vi "Clear Connections.vi"(8 "error in (no error)":errorcluster, 11 "RT Data Cluster in":T1={"Timekeeper hdl"="", "clkDisc session"=variant, "Compiled Data"={"SyncMod?"=FALSE, "SyncMod"="", "ConnectionSettings"={"Mode"=enum."Generate sample clock", "pxitrig"=FALSE, "pfi0"=FALSE, "pfi1"=FALSE, "pfi2"=FALSE, "External Pin"=enum."PFI0", "Routes"=[]}, "TimeKeeper"="", "ScanOffset(%)"=0.0, "StartDelay(s)"=0, "Time Ref Settings"={"Time Reference"=enum."GPS", "Priority 1"=0, "Priority 2"=0, "IRIG type"=enum."IRIGB AM", "Terminal"="", "PPSSetTime"=FALSE, "Start Time"=timestamp(0 s since 1904-01-01)}, "FIFO Locations"={"BoardTime"=[], "Status"=[]}}, "OutputsData"=[], "OutputsFIFO"=refnum, "Scan Period"=0, "Timekeeper type"=enum."6683", "SyncMod type"=enum."6683", "SyncMod hdl"="", "Custom Device Name"=""} {"Compiled Data"."Time Ref Settings"."Priority 2" min=0 max=255; "Compiled Data"."Time Ref Settings"."Priority 1" min=0 max=255}) -> (0 "error out":errorcluster, 3 "RT Data Cluster out":T1={"Timekeeper hdl"="", "clkDisc session"=variant, "Compiled Data"={"SyncMod?"=FALSE, "SyncMod"="", "ConnectionSettings"={"Mode"=enum."Generate sample clock", "pxitrig"=FALSE, "pfi0"=FALSE, "pfi1"=FALSE, "pfi2"=FALSE, "External Pin"=enum."PFI0", "Routes"=[]}, "TimeKeeper"="", "ScanOffset(%)"=0.0, "StartDelay(s)"=0, "Time Ref Settings"={"Time Reference"=enum."GPS", "Priority 1"=0, "Priority 2"=0, "IRIG type"=enum."IRIGB AM", "Terminal"="", "PPSSetTime"=FALSE, "Start Time"=timestamp(0 s since 1904-01-01)}, "FIFO Locations"={"BoardTime"=[], "Status"=[]}}, "OutputsData"=[], "OutputsFIFO"=refnum, "Scan Period"=0, "Timekeeper type"=enum."6683", "SyncMod type"=enum."6683", "SyncMod hdl"="", "Custom Device Name"=""} {"Compiled Data"."Time Ref Settings"."Priority 2" min=0 max=255; "Compiled Data"."Time Ref Settings"."Priority 1" min=0 max=255})   [LabVIEW 2020, in "NI Synchronization Engine.lvlib"]
uses:
  NI Synchronization Engine.lvlib
  RT Data Cluster.ctl
  mdevClkDisc.llb/_clkDisc_session.ctl
  Shared/Compiled Data.ctl
  Shared/Connection Settings.ctl
  Shared/Mode.ctl
  Shared/External Pin.ctl
  Shared/Routes.ctl
  Shared/Route.ctl
  Shared/Time Ref Settings.ctl
  Shared/Time Reference.ctl
  Shared/IRIG Type.ctl
  timekeeper type.ctl
  Timekeeper Route Pin.ctl
  Shared/NI Synchronization Shared.lvlib
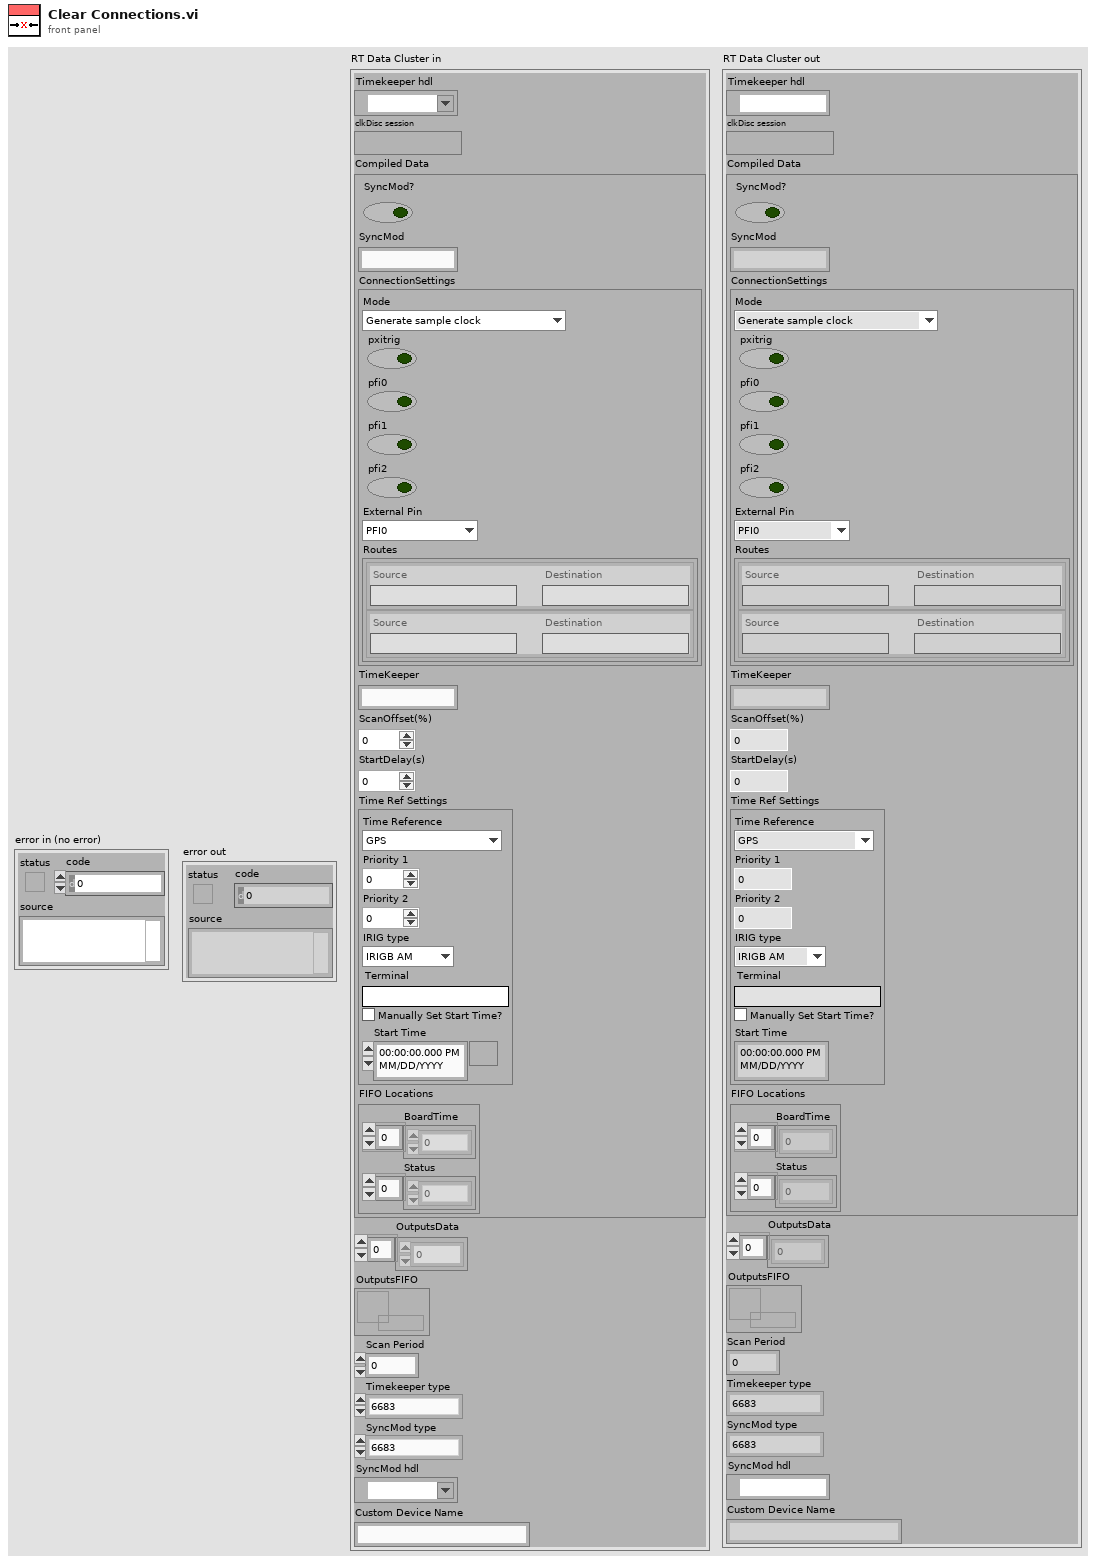
[diagram p1: front panel]
types:
  T1 = typedef "NI Synchronization Engine.lvlib/RT Data Cluster.ctl" = cluster{"Timekeeper hdl":refnum<k15>, "clkDisc session":T2, "Compiled Data":T3, "OutputsData":dbl[], "OutputsFIFO":refnum<k33>, "Scan Period":u32, "Timekeeper type":T12, "SyncMod type":T12, "SyncMod hdl":refnum<k15>, "Custom Device Name":string}
  T2 = typedef "_clkDisc_session.ctl" = variant
  T3 = typedef "NI Synchronization Shared.lvlib/Compiled Data.ctl" = cluster{"SyncMod?":bool, "SyncMod":string, "ConnectionSettings":T4, "TimeKeeper":string, "ScanOffset(%)":dbl, "StartDelay(s)":u16, "Time Ref Settings":T9, "FIFO Locations":cluster{"BoardTime":i32[], "Status":i32[]}}
  T4 = typedef "NI Synchronization Shared.lvlib/Connection Settings.ctl" = cluster{"Mode":T5, "pxitrig":bool, "pfi0":bool, "pfi1":bool, "pfi2":bool, "External Pin":T6, "Routes":T7}
  T5 = typedef "NI Synchronization Shared.lvlib/Mode.ctl" = enum16{"Generate sample clock", "Route sample clock out of chassis", "Route sample clock into chassis", "Custom routes"}
  T6 = typedef "NI Synchronization Shared.lvlib/External Pin.ctl" = enum16{"PFI0", "PFI1", "PFI2"}
  T7 = typedef "NI Synchronization Shared.lvlib/Routes.ctl" = T8[]
  T8 = typedef "NI Synchronization Shared.lvlib/Route.ctl" = cluster{"Source":string, "Destination":string}
  T9 = typedef "NI Synchronization Shared.lvlib/Time Ref Settings.ctl" = cluster{"Time Reference":T10, "Priority 1":i32, "Priority 2":i32, "IRIG type":T11, "Terminal":string, "PPSSetTime":bool, "Start Time":timestamp}
  T10 = typedef "NI Synchronization Shared.lvlib/Time Reference.ctl" = enum16{"GPS", "IRIG", "PPS", "1588 Ordinary Clock", "802.1AS", "PXI Chassis Clock", "Free Running (Internal)"}
  T11 = typedef "NI Synchronization Shared.lvlib/IRIG Type.ctl" = enum16{"IRIGB DC", "IRIGB AM"}
  T12 = typedef "NI Synchronization Engine.lvlib/timekeeper type.ctl" = enum16{"6683", "6683H", "6682", "6682H", "non-timekeeper", "timekeeper"}
  T13 = typedef "NI Synchronization Engine.lvlib/Timekeeper Route Pin.ctl" = enum16{"TTL0", "PFI0", "PFI1", "PFI2", "PXI_Clk10", "PXI_Clk10_In", "BoardClk", "ClkOut", "Oscillator"}
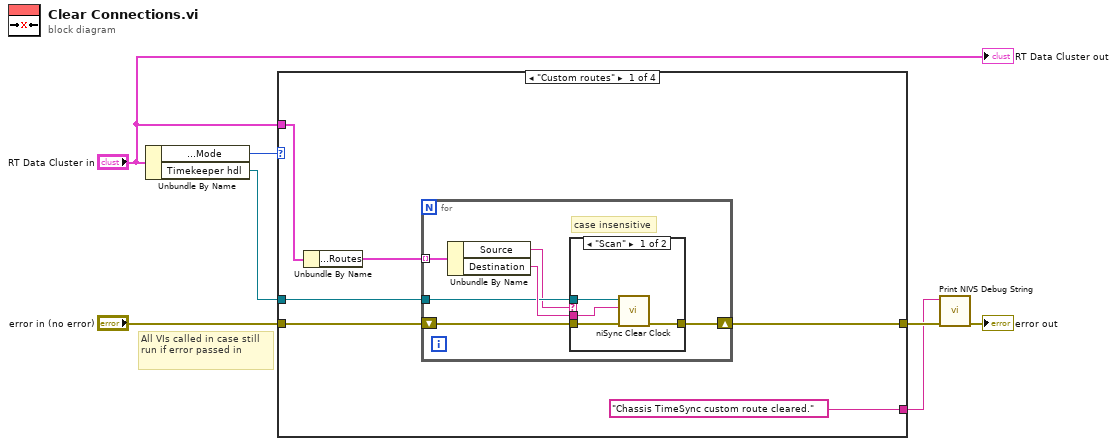
[diagram p0: block diagram]
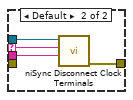
[diagram p2: hidden frame]
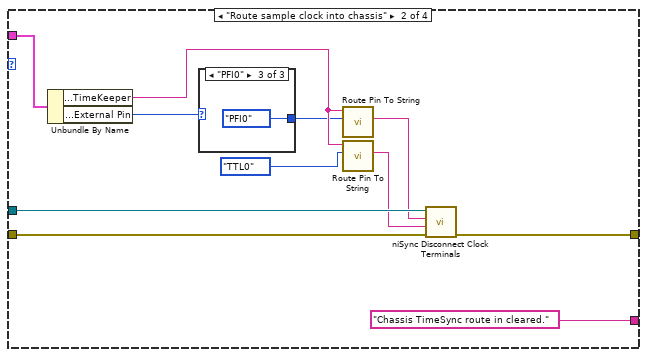
[diagram p3: hidden frame]
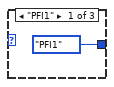
[diagram p4: hidden frame]
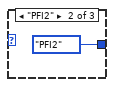
[diagram p5: hidden frame]
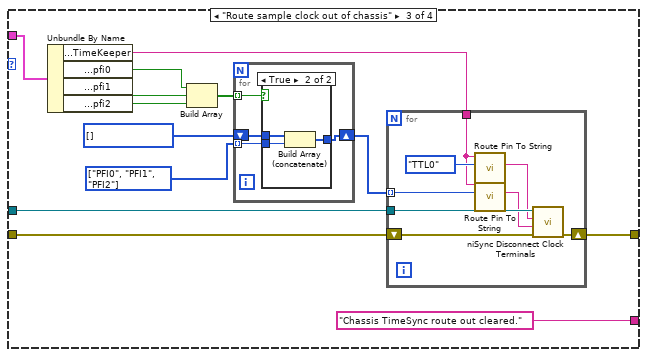
[diagram p6: hidden frame]
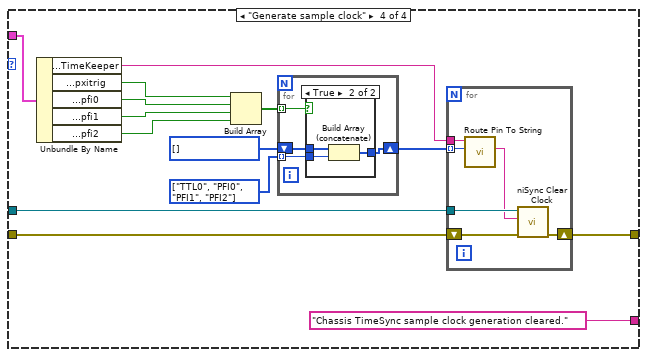
[diagram p8: hidden frame]
diagram:
  # "All VIs called in case still run if error passed in"
  n1 = Unbundle By Name("RT Data Cluster in") -> ("Compiled Data.ConnectionSettings.Mode"=w7:T5, "Timekeeper hdl"=w6:refnum<k15>)
  n2 = case shown="\"Custom routes\"" w7 {
    tunnel: w6 -> [w9 w32 w53 w84]
    tunnel: "RT Data Cluster in" -> [w13 w38 w54 w82]
    tunnel: [w10 w36 w43 w71] -> w4
    tunnel: ["Chassis TimeSync custom route cleared." "Chassis TimeSync route in cleared." "Chassis TimeSync route out cleared." "Chassis TimeSync sample clock generation cleared."] -> w3
    tunnel: "error in (no error)" -> [w8 w28 w42 w72]
    frame "Custom routes" {
      n3 = Unbundle By Name(w13) -> ("Compiled Data.ConnectionSettings.Routes"=w12:T7)
      n4 = for {
        tunnel: w12 -> [w19] mode=indexing
        tunnel: w9 -> [w16]
        shift-right: [w17] -> w10
        shift-left: w8 -> [w14]
        # "case insensitive"
        n5 = Unbundle By Name(w19) -> ("Source"=w15:string, "Destination"=w18:string)
        n6 = case shown="\"Scan\"" w15 {
          selector: w15 -> [_ w24]
          tunnel: w18 -> [w22 w27]
          tunnel: [w23 w26] -> w17
          tunnel: w16 -> [w21 w25]
          tunnel: w14 -> [w20 _]
          frame "Scan" {
            n7 = call <instrlib>:"niSync Clear Clock.vi"("error in (no error)"=w20, "terminal"=w22, "instrument handle"=w21) -> ("error out"=w23:errorcluster)  [unwired: 6 in, 1 out]
          }
          frame Default {
            n8 = call <instrlib>:"niSync Disconnect Clock Terminals.vi"("destination terminal"=w27, "source terminal"=w24, "instrument handle"=w25) -> ("error out"=w26:errorcluster)  [unwired: 7 in, 1 out]
          }
        }
      }
    }
    frame "Route sample clock into chassis" {
      n9 = Unbundle By Name(w38) -> ("Compiled Data.TimeKeeper"=w35:string, "Compiled Data.ConnectionSettings.External Pin"=w37:T6)
      n10 = case shown="\"PFI0\"" w37 {
        tunnel: [Timekeeper_Route_Pin."PFI1" ("Pin") Timekeeper_Route_Pin."PFI2" ("Pin") Timekeeper_Route_Pin."PFI0" ("Pin")] -> w33
        frame "PFI1" {
        }
        frame "PFI2" {
        }
        frame "PFI0" {
        }
      }
      n11 = call "Route Pin To String.vi"("Pin"=w33, "Module"=w35) -> ("String"=w31:string)  [unwired: 9 in]
      n12 = call "Route Pin To String.vi"("Pin"=Timekeeper_Route_Pin."TTL0", "Module"=w35) -> ("String"=w30:string)  [unwired: 9 in]
      n13 = call <instrlib>:"niSync Disconnect Clock Terminals.vi"("error in (no error)"=w28, "destination terminal"=w30, "source terminal"=w31, "instrument handle"=w32) -> ("error out"=w36:errorcluster)  [unwired: 6 in, 1 out]
    }
    frame "Route sample clock out of chassis" {
      w46 = T13[] [enum."PFI0", enum."PFI1", enum."PFI2"] items=["TTL0", "PFI0", "PFI1", "PFI2", "PXI_Clk10", "PXI_Clk10_In", "BoardClk", "ClkOut", "Oscillator"]
      w47 = T13[] [] items=["TTL0", "PFI0", "PFI1", "PFI2", "PXI_Clk10", "PXI_Clk10_In", "BoardClk", "ClkOut", "Oscillator"]
      n14 = Unbundle By Name(w54) -> ("Compiled Data.TimeKeeper"=w52:string, "Compiled Data.ConnectionSettings.pfi0"=w51:bool, "Compiled Data.ConnectionSettings.pfi1"=w50:bool, "Compiled Data.ConnectionSettings.pfi2"=w49:bool)
      n15 = Build Array(w51, w50, w49) -> (w48:bool[])
      n16 = for {
        tunnel: w48 -> [w58] mode=indexing
        shift-right: [w55] -> w45
        shift-left: w47 -> [w57]
        tunnel: w46 -> [w56] mode=indexing
        n17 = case shown="True" w58 {
          tunnel: w57 -> [w59 w62]
          tunnel: w56 -> [_ w61]
          tunnel: [w59 w60] -> w55
          frame False {
          }
          frame True {
            n18 = Build Array (concatenate)(w62, w61) -> (w60:T13[])
          }
        }
      }
      n19 = for {
        tunnel: w53 -> [w70]
        tunnel: w52 -> [w67]
        tunnel: w45 -> [w65] mode=indexing
        shift-right: [w64] -> w43
        shift-left: w42 -> [w63]
        n20 = call "Route Pin To String.vi"("Pin"=Timekeeper_Route_Pin."TTL0", "Module"=w67) -> ("String"=w69:string)  [unwired: 9 in]
        n21 = call "Route Pin To String.vi"("Pin"=w65, "Module"=w67) -> ("String"=w66:string)  [unwired: 9 in]
        n22 = call <instrlib>:"niSync Disconnect Clock Terminals.vi"("error in (no error)"=w63, "destination terminal"=w66, "source terminal"=w69, "instrument handle"=w70) -> ("error out"=w64:errorcluster)  [unwired: 6 in, 1 out]
      }
    }
    frame "Generate sample clock" {
      w79 = T13[] [enum."TTL0", enum."PFI0", enum."PFI1", enum."PFI2"] items=["TTL0", "PFI0", "PFI1", "PFI2", "PXI_Clk10", "PXI_Clk10_In", "BoardClk", "ClkOut", "Oscillator"]
      w80 = T13[] [] items=["TTL0", "PFI0", "PFI1", "PFI2", "PXI_Clk10", "PXI_Clk10_In", "BoardClk", "ClkOut", "Oscillator"]
      n23 = Unbundle By Name(w82) -> ("Compiled Data.TimeKeeper"=w77:string, "Compiled Data.ConnectionSettings.pxitrig"=w76:bool, "Compiled Data.ConnectionSettings.pfi0"=w75:bool, "Compiled Data.ConnectionSettings.pfi1"=w74:bool, "Compiled Data.ConnectionSettings.pfi2"=w73:bool)
      n24 = Build Array(w76, w75, w74, w73) -> (w81:bool[])
      n25 = for {
        tunnel: w81 -> [w88] mode=indexing
        shift-right: [w85] -> w78
        shift-left: w80 -> [w87]
        tunnel: w79 -> [w86] mode=indexing
        n26 = case shown="True" w88 {
          tunnel: w87 -> [w89 w92]
          tunnel: w86 -> [_ w91]
          tunnel: [w89 w90] -> w85
          frame False {
          }
          frame True {
            n27 = Build Array (concatenate)(w92, w91) -> (w90:T13[])
          }
        }
      }
      n28 = for {
        tunnel: w84 -> [w98]
        tunnel: w78 -> [w97] mode=indexing
        tunnel: w77 -> [w95]
        shift-right: [w94] -> w71
        shift-left: w72 -> [w93]
        n29 = call "Route Pin To String.vi"("Pin"=w97, "Module"=w95) -> ("String"=w96:string)  [unwired: 9 in]
        n30 = call <instrlib>:"niSync Clear Clock.vi"("error in (no error)"=w93, "terminal"=w96, "instrument handle"=w98) -> ("error out"=w94:errorcluster)  [unwired: 6 in, 1 out]
      }
    }
  }
  n31 = call "Print NIVS Debug String.vi"("error in (no error)"=w4, "Debug String"=w3) -> ("error out"=→"error out":errorcluster)  [unwired: 8 in]
  "RT Data Cluster out" <- "RT Data Cluster in"
